vi "Shutdown.vi"(8 "error in (no error)":errorcluster, 11 "NavigatableView in":refnum<class "NavigatableView.lvclass">) -> (0 "error out":errorcluster, 3 "NavigatableView out":refnum<class "NavigatableView.lvclass">)   [LabVIEW 2024, in "NavigatableView.lvclass"]
doc: "Send stop event to stop asynchronous view running."
uses:
  NavigatableView.lvclass
  NavigatableView.lvclass/NavigatableView.ctl
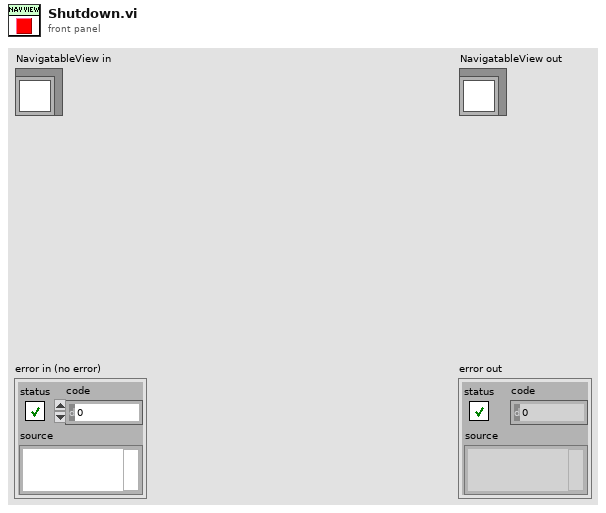
[diagram p1: front panel]
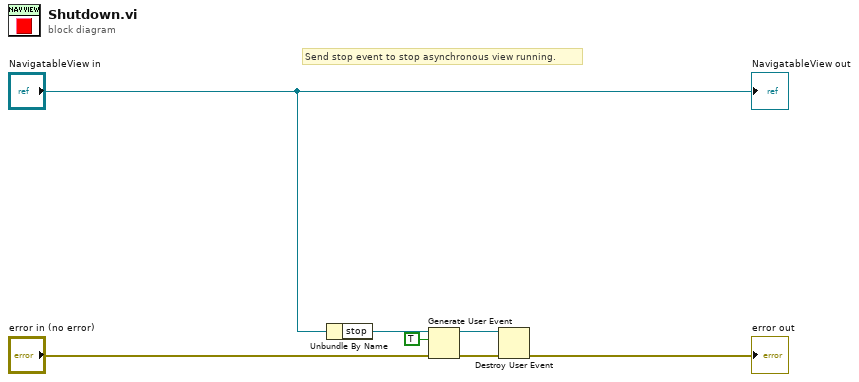
[diagram p0: block diagram]
diagram:
  # "Send stop event to stop asynchronous view running."
  n1 = Unbundle By Name("NavigatableView in") -> ("stop"=w5:refnum<user-event>)
  n2 = Generate User Event(user event=w5, event data cluster=TRUE ("event data"), error in="error in (no error)") -> (user event out=w6:refnum<user-event>, error out=w3:errorcluster)  [unwired: 1 in]
  n3 = Destroy User Event(user event=w6, error in=w3) -> (error out=→"error out":errorcluster)
  "NavigatableView out" <- "NavigatableView in"
